vi "VM3 - 1D Array of Strings.vi"(5 "cmd (read)":enum16{"create", "destroy", "write", "read"}(ring)=enum."read", 7 "VC Handle":T2, 8 "error in":errorcluster, 9 "writer ID":u32, 10 "value in":string[](array[string]), 11 "name_spec":string) -> (0 "error out":errorcluster, 1 "stats":T1, 2 "value out":string[](array[string]), 3 "dup name_spec":string)   [LabVIEW 2021]
doc: "This VI manages variables of the <b>1D Array of Strings</b> data type. Refer to the VI Help for more details.\n\n<b>cmd (read)</b> specifies the operation to perform on the variable: create, write, read, or destroy.\n\n<b>VC Handle</b> specifies the handle of the variable context. To operate on a global variable, pass -1 to this input. <b>name_spec</b> is the name specifier of the desired variable; usually, it is merely a variable name (see the VI Help for more options).\n\n<b>value in</b> and <b>value out</b> are the input and output values written to or read from the variable, respectively.\n\n<b>writer ID</b> specifies the Writer ID to be set along with the new value when writing or creating a variable.\n\n<b>stats</b> returns information about the most recent value of the variable, such as its Writer ID, update time, and update counter.\n\n::: CalcExpress Toolkit :::\nCopyright (c) 2000-2026 Konstantin Shifershteyn. All rights reserved."
uses:
  cetypes.llb/VarMan Variable Context Handle.ctl
  cetypes.llb/VarMan Variable Data Statistics.ctl
  cetypes.llb/VarMan Error Code.ctl
  cersrc/celveng32.dll
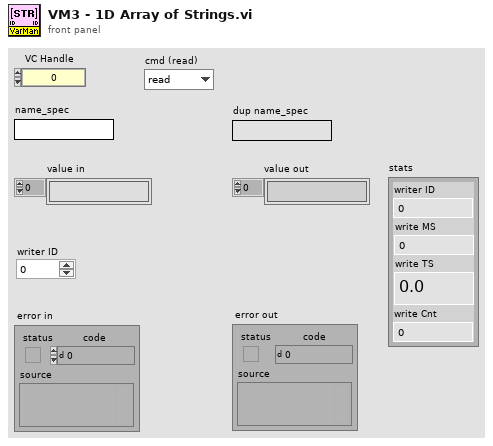
[diagram p1: front panel]
types:
  T1 = typedef "VarMan Variable Data Statistics.ctl" = cluster{"writer ID":u32, "write MS":u32, "write TS":dbl, "write Cnt":u32}
  T2 = typedef "VarMan Variable Context Handle.ctl" = i32
  T3 = enum32{"String", "DBL Number", "identifier", "1D Array of DBL", "2D Array of DBL", "CDB Number", "1D Array of CDB", "2D Array of CDB", "1D Array of String", "2D Array of String", "Unknown data type"}
  T4 = typedef "VarMan Error Code.ctl" = u16
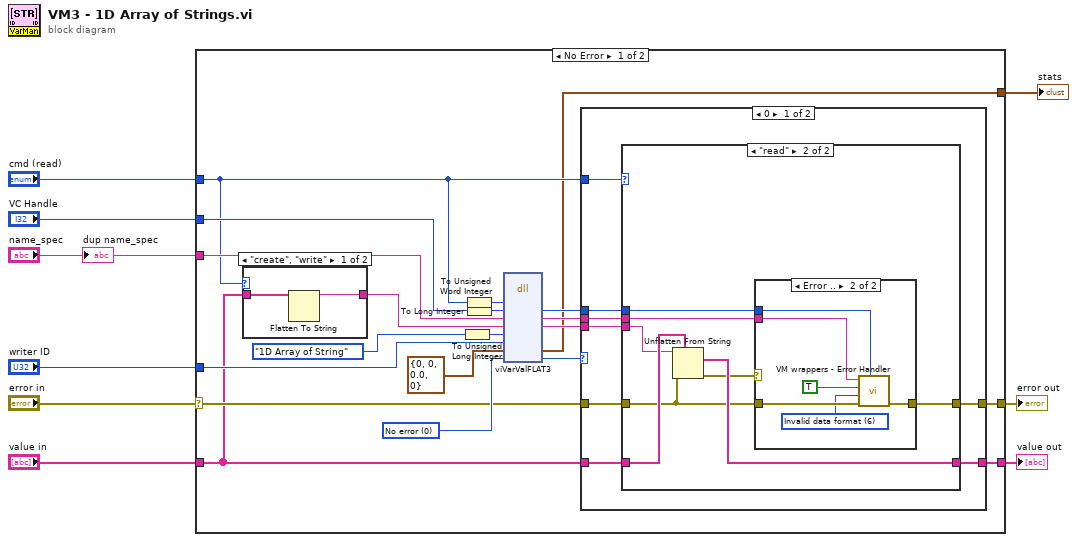
[diagram p0: block diagram]
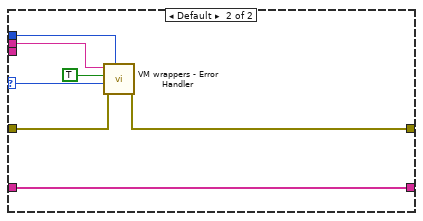
[diagram p5: hidden frame]
diagram:
  n1 = case shown="No Error" "error in" {
    selector: "error in" -> [w21 w65]
    tunnel: [w29 w65] -> w2
    tunnel: "value in" -> [w13 w64]
    tunnel: "name_spec" -> [w28 _]
    tunnel: "VC Handle" -> [w27 _]
    tunnel: [w16 w64] -> w3
    tunnel: "writer ID" -> [w26 _]
    tunnel: "cmd (read)" -> [w15 _]
    tunnel: [w10 _] -> w1
    frame No Error {
      w25 = T4 0 items=["No error", "Invalid variable type", "Variable not found", "Variable already exists", "Invalid context handle", "Input error", "Invalid data format", "No history attached", "History already attached", "Invalid history parameters", "Wrong variable name", "Wrong alias name", "Non-unique alias", "Alias not found", "No alias associated", "Alias already associated", "Wrong context name", "Non-unique context name", "Context name not found", "Invalid parameter", "Generic error", "Memory Full", "Unrecognized LV error", "Unknown error code"] ("VarMan error")
      n2 = case shown="\"create\", \"write\"" w15 {
        tunnel: [w31 _] -> w14
        tunnel: w13 -> [w30 _]
        frame "create", "write" {
          n3 = Flatten To String(anything=w30) -> (data string=w31:string)  [unwired: 3 in, 2 out]
        }
        frame Default {
        }
      }
      n4 = To Unsigned Long Integer(number=T3."1D Array of String" ("data type")) -> (unsigned 32bit integer=w17:u32)
      n5 = To Unsigned Word Integer(number=w15) -> (unsigned 16bit integer=w20:u16)
      n6 = To Long Integer(number=w27) -> (32bit integer=w19:T2)
      n7 = dll-call lib="C:/LV Projects/CalcExpress 40 LV2021/vi.lib/addons/CalcExpress/cersrc/celveng*.dll" fn="viVarValFLAT3"("cmd"=w20, "vch"=w19, "name"=w28, "val"=w14, "type"=w17, "writerID"=w26, "wrStats"=T1 {"writer ID"=0, "write MS"=0, "write TS"=0.0, "write Cnt"=0} ("stats"), "errc"=w25) -> ("vch"=w22:i32, "name"=w23:string, "val"=w12:string, "wrStats"=w10:T1, "errc"=w24:T4)  [unwired: 7 in, 2 out]
      n8 = case shown="0" w24 {
        selector: w24 -> [_ w60]
        tunnel: [w37 w63] -> w29
        tunnel: w21 -> [w38 w62]
        tunnel: w23 -> [w32 w59]
        tunnel: w22 -> [w33 w58]
        tunnel: w15 -> [w39 _]
        tunnel: [w35 w57] -> w16
        tunnel: w13 -> [w36 w57]
        tunnel: w12 -> [w34 _]
        frame 0 {
          n9 = case shown="\"read\"" w39 {
            tunnel: w38 -> [w41 w46]
            tunnel: [w41 w43] -> w37
            tunnel: w36 -> [w40 w49]
            tunnel: [w40 w48] -> w35
            tunnel: w34 -> [_ w47]
            tunnel: w33 -> [_ w45]
            tunnel: w32 -> [_ w44]
            frame Default {
            }
            frame "read" {
              n10 = Unflatten From String(type=w49, binary string=w47, error in (no error)=w46) -> (value=w48:string[], error out=w42:errorcluster)  [unwired: 2 in, 1 out]
              n11 = case shown="Error .." w42 {
                tunnel: w46 -> [w50 w55]
                tunnel: w45 -> [_ w53]
                tunnel: w44 -> [_ w52]
                tunnel: [w50 w51] -> w43
                frame No Error {
                }
                frame Error {
                  w54 = T4 6 items=["No error", "Invalid variable type", "Variable not found", "Variable already exists", "Invalid context handle", "Input error", "Invalid data format", "No history attached", "History already attached", "Invalid history parameters", "Wrong variable name", "Wrong alias name", "Non-unique alias", "Alias not found", "No alias associated", "Alias already associated", "Wrong context name", "Non-unique context name", "Context name not found", "Invalid parameter", "Generic error", "Unknown error code"] ("VarMan error")
                  n12 = call "VM wrappers - Error Handler.vi"("VC Handle"=w53, "error before"=w55, "VarMan error"=w54, "show name spec (F)"=TRUE, "name spec"=w52) -> ("error out"=w51:errorcluster)  [unwired: 5 in, 1 out]
                }
              }
            }
          }
        }
        frame Default {
          n13 = call "VM wrappers - Error Handler.vi"("VC Handle"=w58, "error before"=w62, "VarMan error"=w60, "show name spec (F)"=TRUE, "name spec"=w59) -> ("error out"=w63:errorcluster)  [unwired: 5 in, 1 out]
        }
      }
    }
    frame Error {
    }
  }
  "value out" <- w3
  "error out" <- w2
  "stats" <- w1
  "dup name_spec" <- "name_spec"
